vi "Create Abstracted Reader.vi"(6 "Timeout (ms)":u32=5000, 7 "Element Alignment":u32, 8 "error in (no error)":errorcluster, 9 "Array":bool, 10 "Topic Name":T1, 11 "Element Size":u32) -> (0 "error out":errorcluster, 3 "Reader Reference":T2 {"refnum" format="%.0x"})   [LabVIEW 2021, in "Iceoryx.lvlib"]
doc: "Create a reader using abstract data. The normal create detects the topic information dynamically. This will accept the abstract data instead of detecting it."
uses:
  Refnum/Typedef/BB Reader Refnum.ctl
  typedef/Topic Full Names.ctl
  typedef/Errors.ctl
  SubVIs/Add Error Core.vi
  <vilib>/CIF Foundation/CIF Utilities/File/SubVIs/File Not Found Error Core.vi
  SubVIs/Convert Error Core.vi
  Iceoryx.lvlib
  <vilib>/CIF Foundation/CIF Utilities/File/File_CIF_U.lvlib
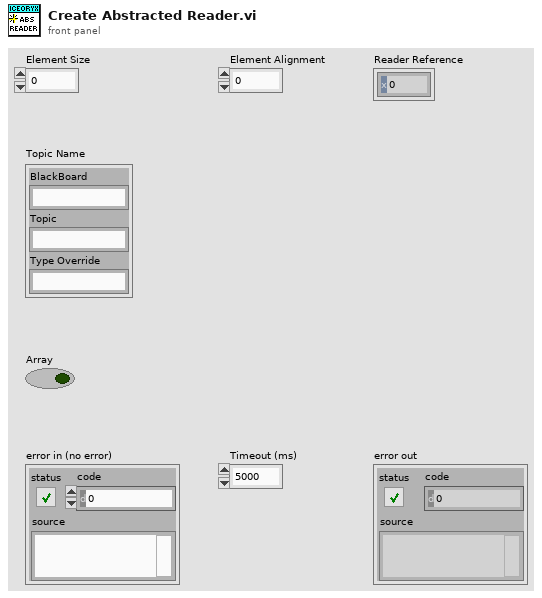
[diagram p1: front panel]
types:
  T1 = typedef "Iceoryx.lvlib/Topic Full Names.ctl" = cluster{"BlackBoard":string, "Topic":string, "Type Override":string}
  T2 = typedef "Iceoryx.lvlib/BB Reader Refnum.ctl" = cluster{"refnum":u64, "BB Reader":enum8{"bb_reader"}}
  T3 = typedef "Iceoryx.lvlib/Errors.ctl" = enum16{"Unsupported Type", "Empty Name", "Cluster Name"}
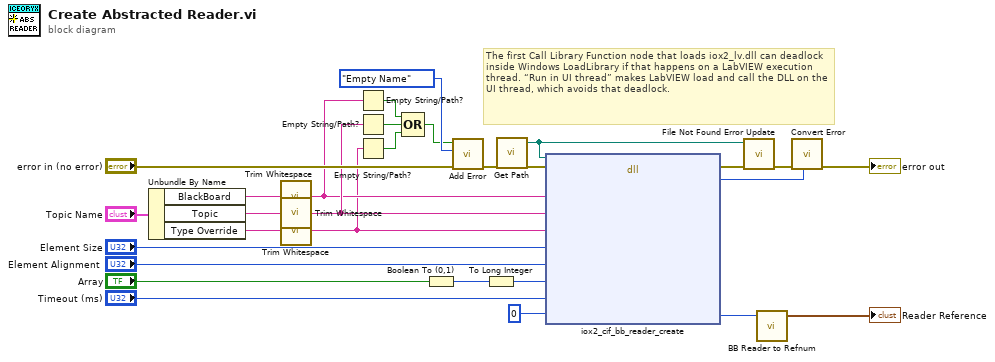
[diagram p0: block diagram]
diagram:
  # "The first Call Library Function node that loads iox2_lv.dll can deadlock inside Windows LoadLibrary if that happens on a LabVIEW execution thread. “Run in UI thread” makes LabVIEW load and call the DLL on the UI thread, which avoids that deadlock."
  n1 = Unbundle By Name("Topic Name") -> ("BlackBoard"=w12:string, "Topic"=w11:string, "Type Override"=w10:string)
  n2 = call <vilib>:"Trim Whitespace.vi"("string"=w12) -> ("trimmed string"=w14:string)  [unwired: 1 in]
  n3 = call <vilib>:"Trim Whitespace.vi"("string"=w11) -> ("trimmed string"=w15:string)  [unwired: 1 in]
  n4 = call <vilib>:"Trim Whitespace.vi"("string"=w10) -> ("trimmed string"=w1:string)  [unwired: 1 in]
  n5 = Empty String/Path?(string/path=w14) -> (empty?=w17:bool)
  n6 = Empty String/Path?(string/path=w15) -> (empty?=w18:bool)
  n7 = Empty String/Path?(string/path=w1) -> (empty?=w2:bool)
  n8 = Compound Arithmetic op=OR(w17, w18, w2) -> (w16:bool)
  n9 = Boolean To (0,1)(Boolean="Array") -> (0, 1=w9:i16)
  n10 = call "Add Error.vi"("error in (no error)"="error in (no error)", "Error"=Errors."Empty Name", "Insert Error"=w16) -> ("error out"=w3:errorcluster)  [unwired: 8 in]
  n11 = To Long Integer(number=w9) -> (32bit integer=w8:i32)
  n12 = call "Get Path.vi"() -> ("libiox2_cif path"=w24:path)  [unwired: 4 in]
  n13 = dll-call lib="D:/dev/iceoryx2_lvwrapper/dist/iox2_cif.dll" fn="iox2_cif_bb_reader_create"(path in=w24, error in=w3, "bb_name"=w14, "topic"=w15, "type_name"=w1, "elem_size"="Element Size", "elem_align"="Element Alignment", "is_iox2_cif_array"=w8, "timeout_ms"="Timeout (ms)", "reader"=u64 0 ("writer")) -> (error out=w23:errorcluster, "return type"=w22:i32, "reader"=w28:u64)  [unwired: 8 in, 1 out]
  n14 = call <vilib>:"File Not Found Error Update.vi"("error in"=w23, "path in"=w24) -> ("error out"=w25:errorcluster)  [unwired: 9 in]
  n15 = call "BB Reader to Refnum.vi"("BB Reader U64"=w28) -> ("BB Reader Refnum"=→"Reader Reference":T2)  [unwired: 4 in]
  n16 = call "Convert Error.vi"("return type"=w22, "error in (no error)"=w25) -> ("error out"=→"error out":errorcluster)  [unwired: 9 in]
